vi "[ce] Eval X-Y-Z(a,t1,t2).vi"(6 "parameters":cluster{"name":string, "value":dbl}[](array[cluster]) {"value" format="%.2f"}, 7 "# points":u32=25, 8 "error in":errorcluster, 9 "formulas info":T1, 10 "End":cluster{"t1":dbl, "t2":dbl}={"t1"=1.0, "t2"=1.0} {"t2" format="%.2f"; "t1" format="%.2f"}, 11 "Start":cluster{"t1":dbl, "t2":dbl} {"t2" format="%.2f"; "t1" format="%.2f"}) -> (0 "error out":errorcluster, 1 "Z(t1,t2)":dbl[](array[numeric]) format="%.2f", 2 "Y(t1,t2)":dbl[](array[numeric]) format="%.2f", 3 "X(t1,t2)":dbl[](array[numeric]) format="%.2f", 4 "ticks":u32)   [LabVIEW 2021]
doc: "Describes a surface in 3D with two variables running over two different intervals. In addition, the VI allows specifying additional parameters and evaluating them in formulas.\n\n::: CalcExpress Toolkit :::\nCopyright (c) 2000-2026 Konstantin Shifershteyn. All rights reserved."
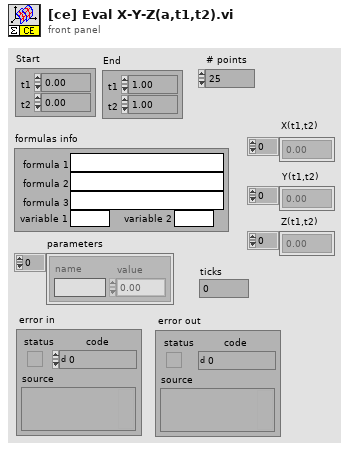
[diagram p1: front panel]
types:
  T1 = cluster{"formula 1":string, "formula 2":string, "formula 3":string, "variable 1":string, "variable 2":string}
  T2 = enum16{"create", "destroy", "set value", "get value"}
  T3 = typedef "VarMan Variable Context Handle.ctl" = i32
  T4 = cluster{"formula 3":string, "variable 1":string, "variable 2":string}
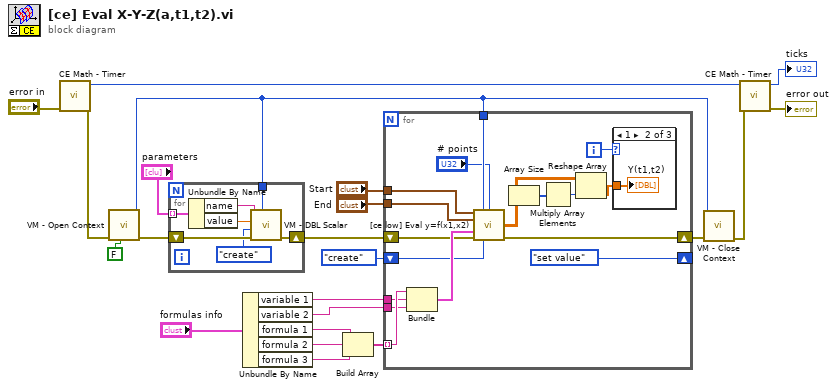
[diagram p0: block diagram]
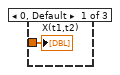
[diagram p2: hidden frame]
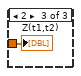
[diagram p3: hidden frame]
diagram:
  n1 = call "CE Math - Timer.vi"("error in (no error)"="error in") -> ("error out"=w21:errorcluster, "ticks out"=w22:u32)  [unwired: 7 in]
  n2 = call "VM - Open Context.vi"("close loose contexts (F)"=FALSE ("close loose contexts (T)"), "error in"=w21) -> ("error out"=w17:errorcluster, "VC Handle out"=w13:T3)  [unwired: 7 in, 1 out]
  n3 = for {
    shift-right: [w26] -> w3
    shift-left: w17 -> [w27]
    tunnel: "parameters" -> [w24] mode=indexing
    tunnel: w13 -> [w23]
    n4 = Unbundle By Name(w24) -> ("name"=w28:string, "value"=w29:dbl)
    n5 = call "VM - DBL Scalar.vi"("VC Handle"=w23, "error in"=w27, "cmd"=T2."create", "value in"=w29, "name_spec"=w28) -> ("error out"=w26:errorcluster)  [unwired: 1 in, 5 out]
  }
  n6 = Unbundle By Name("formulas info") -> ("variable 1"=w10:string, "variable 2"=w9:string, "formula 1"=w7:string, "formula 2"=w8:string, "formula 3"=w6:string)
  n7 = Build Array(w7, w8, w6) -> (w5:string[])
  n8 = for {
    tunnel: w13 -> [w41]
    tunnel: "Start" -> [w39]
    tunnel: "End" -> [w38]
    tunnel: w10 -> [w30]
    tunnel: w9 -> [w31]
    tunnel: w5 -> [w32] mode=indexing
    shift-right: [w33] -> w2
    shift-left: w3 -> [w36]
    shift-right: [T2."set value" ("vm cmd")] -> _
    shift-left: T2."create" ("vm cmd") -> [w35]
    i -> [w46]
    n9 = Bundle("formula 3"=w32, "variable 1"=w30, "variable 2"=w31) -> (w37:T4)  [unwired: 1 in]
    n10 = call "[ce low] Eval y=f(x1,x2).vi"("Start"=w39, "VC Handle"=w41, "number of points"="# points", "End"=w38, "formula info"=w37, "error in"=w36, "vm cmd"=w35) -> ("Y Values"=w43:dbl[][], "error out"=w33:errorcluster)  [unwired: 5 in, 2 out]
    n11 = Array Size(array=w43) -> (size(s)=w44:i32[])
    n12 = Multiply Array Elements(1:w44) -> (0:w45:i32)
    n13 = Reshape Array(w43, w45) -> (w42:dbl[])
    n14 = case shown="1" w46 {
      tunnel: w42 -> [w47 w48 w49]
      frame 0, Default {
        "X(t1,t2)" <- w47
      }
      frame 1 {
        "Y(t1,t2)" <- w48
      }
      frame 2 {
        "Z(t1,t2)" <- w49
      }
    }
  }
  n15 = call "VM - Close Context.vi"("error in"=w2, "VC Handle"=w13) -> ("error out"=w19:errorcluster)  [unwired: 8 in, 1 out]
  n16 = call "CE Math - Timer.vi"("error in (no error)"=w19, "ticks in"=w22) -> ("error out"=→"error out":errorcluster, "ticks out"=→"ticks":u32)  [unwired: 6 in]
